vi "Calculate Load Values.vi"(0 "DAC HeatFlow AIV in":refnum<class "DAC HeatFlow AIV.lvclass">, 7 "U Load":dbl, 11 "error in":errorcluster) -> (4 "DAC HeatFlow AIV out":refnum<class "DAC HeatFlow AIV.lvclass">, 12 "P teg":dbl, 13 "I Load":dbl, 14 "U Load":dbl, 15 "error out":errorcluster)   [LabVIEW 2019, in "DAC.lvlib" / "DAC HeatFlow AIV.lvclass"]
uses:
  DAC HeatFlow AIV.lvclass
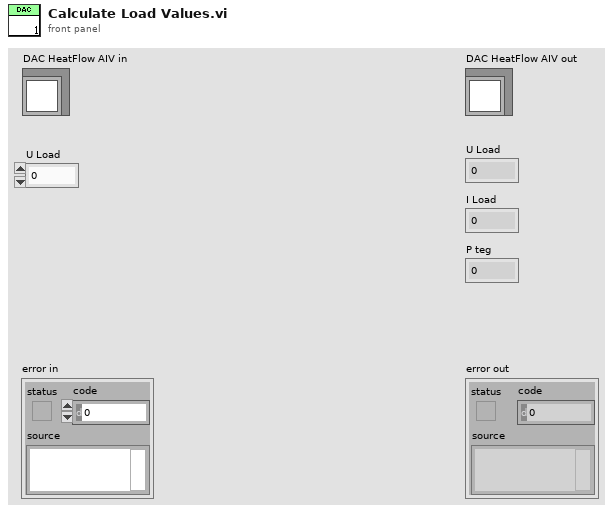
[diagram p1: front panel]
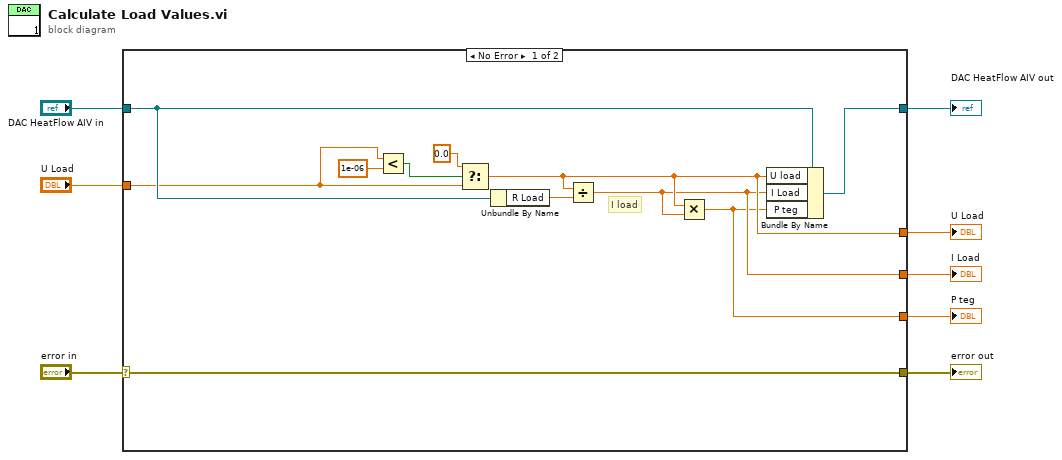
[diagram p0: block diagram]
diagram:
  n1 = case shown="No Error" "error in" {
    selector: "error in" -> [w19 w21]
    tunnel: [w19 w21] -> w7
    tunnel: [w12 w20] -> w5
    tunnel: "DAC HeatFlow AIV in" -> [w15 w20]
    tunnel: "U Load" -> [w14 _]
    tunnel: [w11 _] -> w3
    tunnel: [w10 _] -> w2
    tunnel: [w9 _] -> w1
    frame No Error {
      # "I load"
      n2 = Less?(x=w14, y=1e-06) -> (x < y?=w17:bool)
      n3 = Select(t=0.0, s=w17, f=w14) -> (s? t:f=w11:dbl)
      n4 = Unbundle By Name(w15) -> ("R Load"=w13:dbl)
      n5 = Divide(x=w11, y=w13) -> (x/y=w10:dbl)
      n6 = Multiply(x=w11, y=w10) -> (x*y=w9:dbl)
      n7 = Bundle By Name(cluster=w15, "U load"=w11, "I Load"=w10, "P teg"=w9) -> (w12:refnum<class "DAC HeatFlow AIV.lvclass">)
    }
    frame Error {
    }
  }
  "error out" <- w7
  "DAC HeatFlow AIV out" <- w5
  "U Load" <- w3
  "I Load" <- w2
  "P teg" <- w1
